vi "Coarse Timing Synchronization.vi"(11 "Array":cdb[](array[numeric])) -> (1 "max value":dbl, 2 "Coarse packet est":dbl)   [LabVIEW 2024]
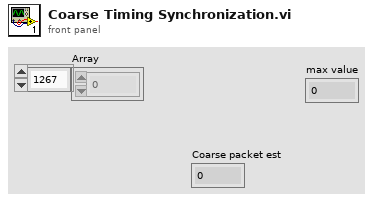
[diagram p1: front panel]
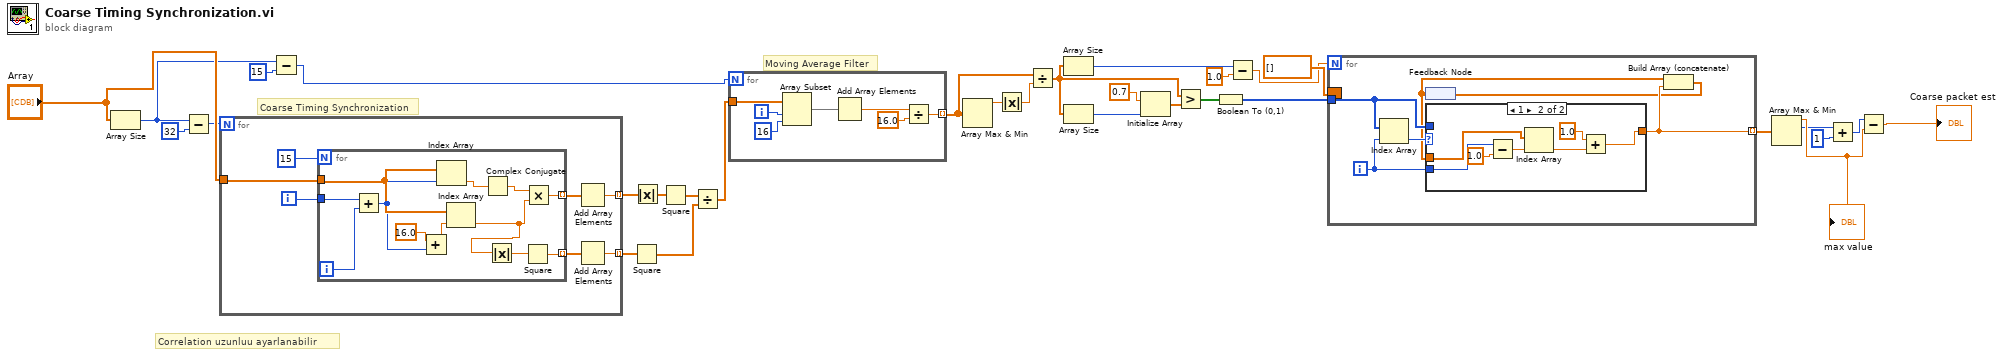
[diagram p0: block diagram]
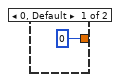
[diagram p2: hidden frame]
diagram:
  # "Correlation uzunluu ayarlanabilir"
  # "Moving Average Filter"
  # "Coarse Timing Synchronization"
  n1 = Array Size(array="Array") -> (size(s)=w26:i32)
  n2 = Subtract(x=w26, y=32) -> (x-y=w2:i32)
  n3 = for {
    N: w2 -> [_]
    tunnel: "Array" -> [w37]
    tunnel: [w33] -> w4 mode=indexing
    tunnel: [w32] -> w5 mode=indexing
    i -> [w36]
    n4 = for {
      N: 15 -> [_]
      tunnel: w37 -> [w49]
      tunnel: w36 -> [w47]
      tunnel: [w44] -> w35 mode=indexing
      tunnel: [w43] -> w34 mode=indexing
      i -> [w48]
      n5 = Add(x=w47, y=w48) -> (x+y=w42:i32)
      n6 = Add(x=16.0, y=w42) -> (x+y=w45:dbl)
      n7 = Index Array(array=w49, index=w42) -> (element=w39:cdb)
      n8 = Index Array(array=w49, index=w45) -> (element=w41:cdb)
      n9 = Complex Conjugate(1:w39) -> (0:w40:cdb)
      n10 = Absolute Value(x=w41) -> (abs(x)=w50:dbl)
      n11 = Square(x=w50) -> (x^2=w44:dbl)
      n12 = Multiply(x=w40, y=w41) -> (x*y=w43:cdb)
    }
    n13 = Add Array Elements(numeric array=w34) -> (sum=w33:cdb)
    n14 = Add Array Elements(numeric array=w35) -> (sum=w32:dbl)
  }
  n15 = Subtract(x=w26, y=15) -> (x-y=w10:i32)
  n16 = Square(x=w5) -> (x^2=w7:dbl[])
  n17 = Absolute Value(x=w4) -> (abs(x)=w3:dbl[])
  n18 = Square(x=w3) -> (x^2=w6:dbl[])
  n19 = Divide(x=w6, y=w7) -> (x/y=w8:dbl[])
  n20 = for {
    N: w10 -> [_]
    tunnel: w8 -> [w55]
    tunnel: [w51] -> w13 mode=indexing
    i -> [w56]
    n21 = Array Subset(array=w55, index=w56, length=16) -> (w54:dbl[])
    n22 = Add Array Elements(numeric array=w54) -> (sum=w53:dbl)
    n23 = Divide(x=w53, y=16.0) -> (x/y=w51:dbl)
  }
  n24 = Array Max & Min(array=w13) -> (max value=w12:dbl)  [unwired: 3 out]
  n25 = Absolute Value(x=w12) -> (abs(x)=w11:dbl)
  n26 = Divide(x=w13, y=w11) -> (x/y=w19:dbl[])
  n27 = Array Size(array=w19) -> (size(s)=w21:i32)
  n28 = Array Size(array=w19) -> (size(s)=w14:i32)
  n29 = Initialize Array(0.7 ("element"), w14) -> (w16:dbl[])
  n30 = Greater?(x=w19, y=w16) -> (0:w27:bool[])
  n31 = Boolean To (0,1)(Boolean=w27) -> (0, 1=w20:i16[])
  n32 = Subtract(x=w21, y=1.0) -> (x-y=w17:dbl)
  n33 = for {
    N: w17 -> [_]
    tunnel: w20 -> [w62]
    tunnel: [w60] -> w23 mode=indexing
    border: dbl[] [] -> [_]
    i -> [w61]
    n34 = Index Array(array=w62, index=w61) -> (element=w63:i16)
    n35 = feedback #1() -> (w58:dbl[])
    n36 = case shown="1" w63 {
      tunnel: w61 -> [_ w66]
      tunnel: w62 -> [_ _]
      tunnel: [0 w69] -> w60
      tunnel: w58 -> [_ w68]
      frame 0, Default {
      }
      frame 1 {
        n37 = Subtract(x=w66, y=1.0) -> (x-y=w65:dbl)
        n38 = Index Array(array=w68, index=w65) -> (element=w71:dbl)
        n39 = Add(x=1.0, y=w71) -> (x+y=w69:dbl)
      }
    }
    n40 = Build Array (concatenate)(w58, w60) -> (w59:dbl[])
    n41 = feedback-in #1(w59) -> ()
  }
  n42 = Array Max & Min(array=w23) -> (max value=w30:dbl, max index (indices)=w24:i32)  [unwired: 2 out]
  "max value" <- w30
  n43 = Add(x=w24, y=1) -> (x+y=w29:i32)
  n44 = Subtract(x=w29, y=w30) -> (x-y=→"Coarse packet est":dbl)
